vi "SPARK Clear Faults.vi"(8 "error in":errorcluster, 11 "Spark refnum":T1) -> (0 "error out":errorcluster, 3 "Spark refnum":T1)   [LabVIEW 2023, in "REVLibDriver.lvlib"]
doc: "Clear the device sticky faults and warnings"
uses:
  <vilib>/REVLibDriver/REVLibDriver.lvlib
  <vilib>/REV Custom Controls/REVSparkRefnum.ctl
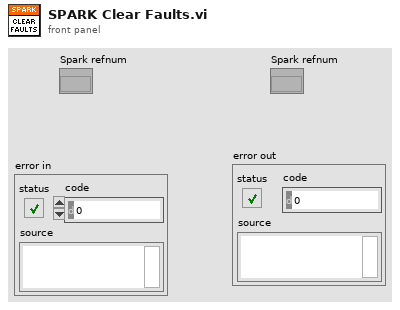
[diagram p1: front panel]
types:
  T1 = typedef "REVLibDriver.lvlib/REVSparkRefnum.ctl" = refnum<k20>
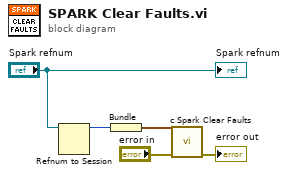
[diagram p0: block diagram]
diagram:
  n1 = Refnum to Session(7:"Spark refnum") -> (3:w3:u64)  [unwired: 1 in, 1 out]
  n2 = Bundle("Session"=w3) -> (w1:cluster{"Session":u64})  [unwired: 1 in]
  n3 = call <vilib>:"c Spark Clear Faults.vi"("error in (no error)"="error in", "handle"=w1) -> ("error out"=→"error out":errorcluster)  [unwired: 7 in, 2 out]
  "Spark refnum" <- "Spark refnum"
